vi "RDV-handle-findmeasurementparameter.vi"(8 "error in (no error)":errorcluster, 11 "RDV-Reflection_Data_viewer in":refnum<class "RDV-Reflection_Data_viewer.lvclass">) -> (0 "error out":errorcluster, 2 "Measurement Parameter":T1[](array[typedef]) {"lenght" format="%#_6p"; "cap" format="%#_6p"; "Tau" format="%#_6p"}, 3 "RDV-Reflection_Data_viewer out":refnum<class "RDV-Reflection_Data_viewer.lvclass">)   [LabVIEW 2020, in "RDV-Reflection_Data_viewer.lvclass"]
doc: "Finds Tau, capacitance and length for every data set in the viewer's map and returns them per name."
uses:
  RDV-Reflection_Data_viewer.lvclass
  RDV-INFO_DATA.ctl
  Computation/RDC-Probe_parameters.ctl
  Computation/RDC-Reflection_Data_Computation.lvlib
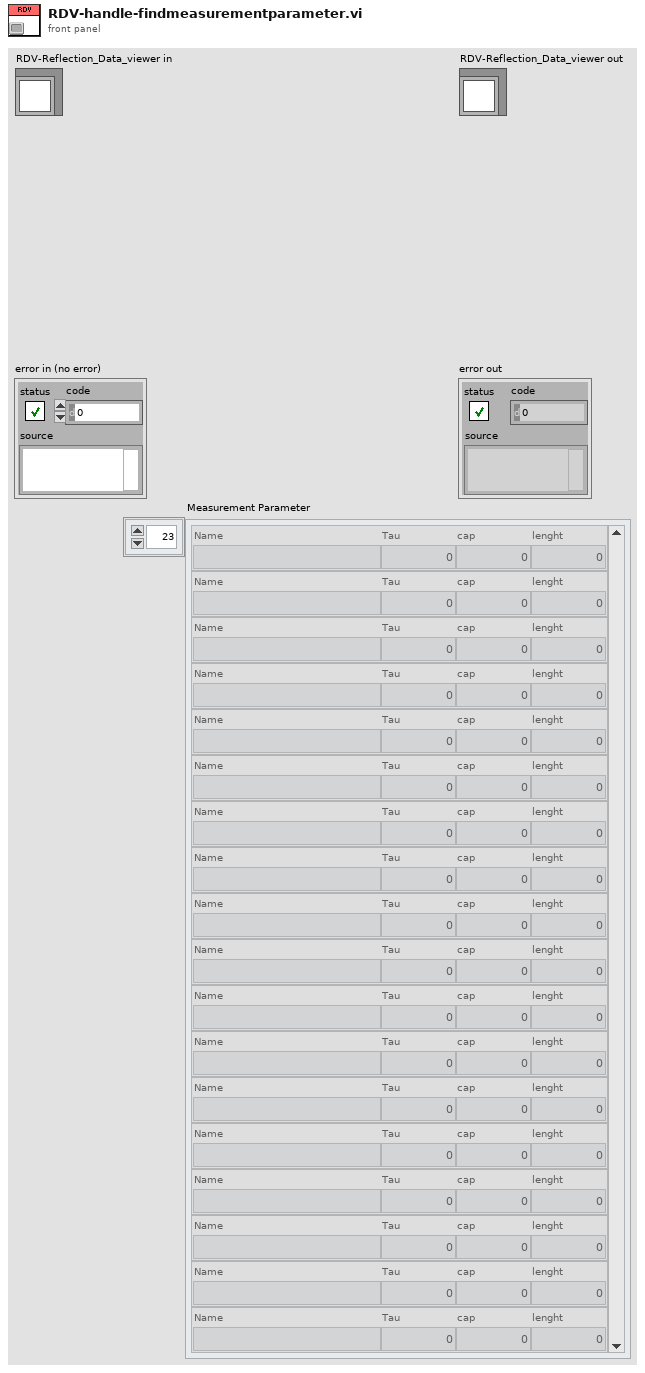
[diagram p1: front panel]
types:
  T1 = typedef "RDV-Reflection_Data_viewer.lvclass/RDV-INFO_DATA.ctl" = cluster{"Name":string, "Tau":dbl, "cap":dbl, "lenght":dbl}
  T2 = typedef "RDC-Reflection_Data_Computation.lvlib/RDC-Probe_parameters.ctl" = cluster{"lenght [mm]":dbl, "Core Diameter [mm]":dbl, "Inner Diameter [mm]":dbl, "Dieletrisk constant":dbl}
  T3 = typedef "RFH-Reflection_File_Handler.lvlib/RFH-common_data_format.ctl" = cluster{"Frequency":dbl[], "Reflection'":dbl[], "Reflection''":dbl[], "Permativity'":dbl[], "Permativity''":dbl[], "Conductivity":dbl[], "Loss Tangent":dbl[], "Resistance":dbl[], "Reactance":dbl[]}
  T4 = typedef "RDV-Reflection_Data_viewer.lvclass/RDV-DATA_MAP_CLUST.ctl" = cluster{"filename w/ ext":string, "Common Format":T3}
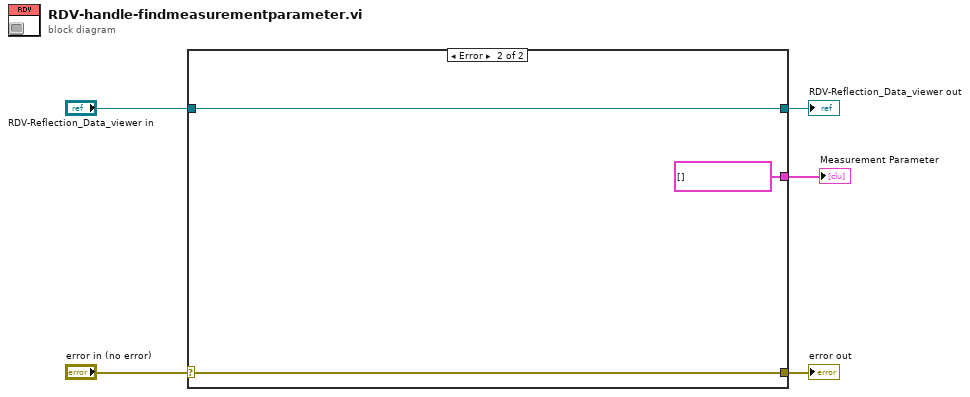
[diagram p0: block diagram]
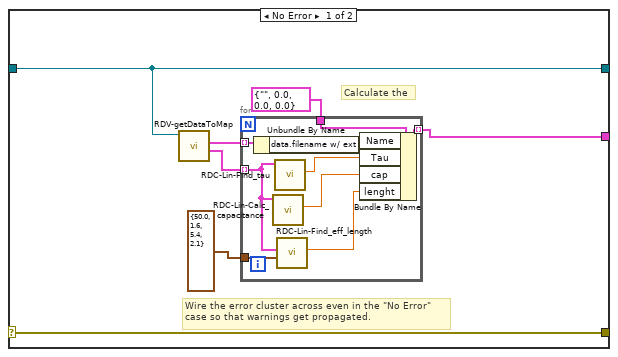
[diagram p2: hidden frame]
diagram:
  n1 = case shown="Error" "error in (no error)" {
    selector: "error in (no error)" -> [w12 w24]
    tunnel: [w12 w24] -> w4
    tunnel: [w7 w23] -> w2
    tunnel: "RDV-Reflection_Data_viewer in" -> [w7 w23]
    tunnel: [w6 T1[] []] -> w1
    frame No Error {
      # "Calculate the"
      # "Wire the error cluster across even in the \"No Error\"\ncase so that warnings get propagated."
      n2 = call "RDV-getDataToMap.vi"("RDV-Reflection_Data_viewer in"=w7) -> ("data"=w9:T3[], "all data"=w10:cluster{"key":string, "data":T4}[])  [unwired: 7 in, 2 out]
      n3 = for {
        tunnel: T1 {"Name"="", "Tau"=0.0, "cap"=0.0, "lenght"=0.0} ("data info") -> [w21]
        tunnel: [w20] -> w6 mode=indexing
        tunnel: w10 -> [w16] mode=indexing
        tunnel: w9 -> [w15] mode=indexing
        tunnel: T2 {"lenght [mm]"=50.0, "Core Diameter [mm]"=1.6, "Inner Diameter [mm]"=5.4, "Dieletrisk constant"=2.1} ("Probe Parameters") -> [w14]
        n4 = Unbundle By Name(w16) -> ("data.filename w/ ext"=w19:string)
        n5 = call "RDC-Lin-Calc_capacitance.vi"("Open Probe reading"=w15) -> ("C0"=w18:dbl)  [unwired: 9 in, 1 out]
        n6 = call "RDC-Lin-Find_tau.vi"("Short Probe reading"=w15) -> ("Tau"=w17:dbl)  [unwired: 9 in, 1 out]
        n7 = call "RDC-Lin-Find_eff_length.vi"("Probe Parameters"=w14, "Short Probe reading"=w15) -> ("Lenght"=w13:dbl)  [unwired: 8 in, 1 out]
        n8 = Bundle By Name(cluster=w21, "Name"=w19, "Tau"=w17, "cap"=w18, "lenght"=w13) -> (w20:T1)
      }
    }
    frame Error {
    }
  }
  "error out" <- w4
  "RDV-Reflection_Data_viewer out" <- w2
  "Measurement Parameter" <- w1
